vi "_CSMOFGV.vi"(6 "Operation":T7=enum."Get By Name", 7 "Allowed Messages (Empty For All)":string[](array[string]), 8 "Error In":errorcluster caption="error in (no error)", 9 "Mode":T1, 10 "Reference":string, 11 "Name (\"\" to Use UUID) In":string) -> (0 "error out":errorcluster, 1 "Boolean":bool, 3 "Array":T2[](array[typedef]))   [LabVIEW 2017, in "Communicable State Machine.lvlib"]
uses:
  Communicable State Machine.lvlib
  _CSMOFGVOPER.ctl
  _CSMObj.ctl
  _CSMObj-Info.ctl
  Typedef/_CSM_MODE.ctl
  _CSMObj-Refs.ctl
  _CSMObj-Data.ctl
  Typedef/_CSM_MSG_TYPE.ctl
  Priority Queue/Priority Queue.ctl
  Typedef/_Cross CSM State Data.ctl
  Typedef/_Cross CSM State Response.ctl
  Typedef/_CSM_Response Source Message.ctl
  Priority Queue/def-Data(LowPRI-Q).ctl
  _CSMObj-ModeData.ctl
  Typedef/_CSM Status Change Event Data.ctl
  Typedef/_CSM_List Module Scope.ctl
  Def-CSMOMgr.ctl
  ChangeFlag/ChangeFlag-Write.vi
  Utility/Random Change Flag.vi
  ChangeFlag/ChangeFlagDB.vi
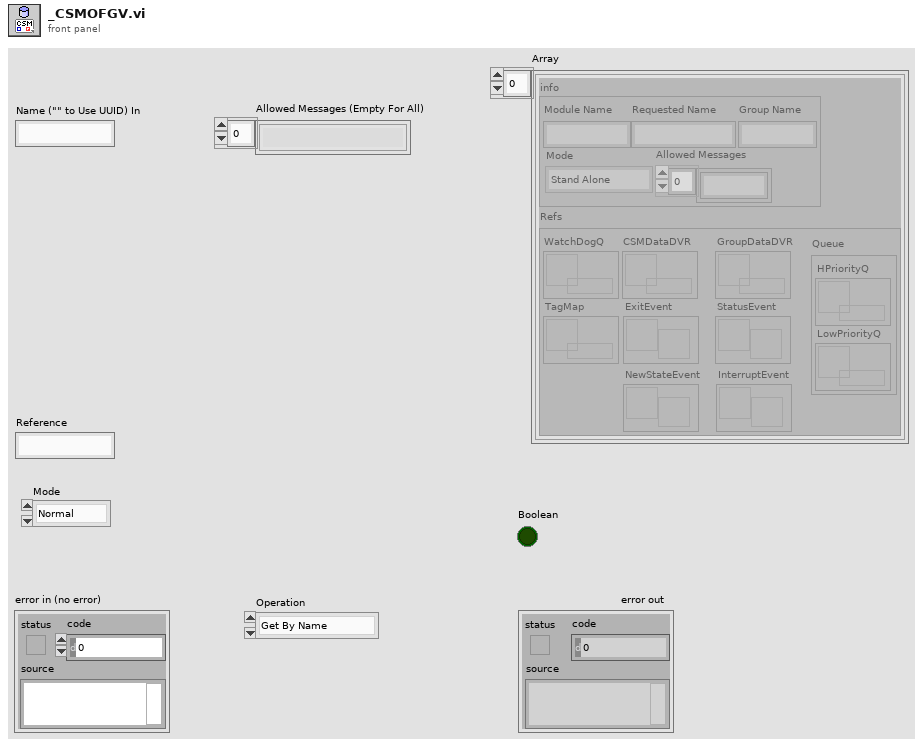
[diagram p1: front panel]
types:
  T1 = typedef "Communicable State Machine.lvlib/_CSM_List Module Scope.ctl" = enum16{"Normal", "System Only", "All"}
  T2 = typedef "Communicable State Machine.lvlib/_CSMObj.ctl" = cluster{"info":T3, "Refs":T5}
  T3 = typedef "Communicable State Machine.lvlib/_CSMObj-Info.ctl" = cluster{"Module Name":string, "Requested Name":string, "Group Name":string, "Mode":T4, "Allowed Messages":string[]}
  T4 = typedef "Communicable State Machine.lvlib/_CSM_MODE.ctl" = enum16{"Not Exist", "Stand Alone", "CSM", "Worker", "Worker Agent", "Chain Node", "Chain"}
  T5 = typedef "Communicable State Machine.lvlib/_CSMObj-Refs.ctl" = cluster{"WatchDogQ":refnum<queue>, "CSMDataDVR":refnum<data-value>, "Queue":T6, "GroupDataDVR":refnum<data-value>, "TagMap":refnum<data-value>, "ExitEvent":refnum<user-event>, "NewStateEvent":refnum<user-event>, "StatusEvent":refnum<user-event>, "InterruptEvent":refnum<user-event>}
  T6 = typedef "Communicable State Machine.lvlib/Priority Queue.ctl" = cluster{"HPriorityQ":refnum<queue>, "LowPriorityQ":refnum<queue>}
  T7 = typedef "Communicable State Machine.lvlib/_CSMOFGVOPER.ctl" = enum16{"Create If not Exist", "Get By Name", "List", "Check If Name Exists", "Release", "Module Status", "Create Status Event Handler", "Destroy Status Event Handler", "Clear Invalid Objs"}
  T8 = typedef "Communicable State Machine.lvlib/Def-CSMOMgr.ctl" = variant
  T9 = typedef "Communicable State Machine.lvlib/_CSMObj-ModeData.ctl" = cluster{"CSMDataDVR":refnum<data-value>[], "PriorityQueues":T6[], "Messages of Chain Nodes":cluster{"Module Name":string, "Allowed Messages":string[]}[], "Chain Message Mapping Map":variant, "SharedRegistryRules":string[]}
  T10 = cluster{"Module Name":string, "Allowed Messages":string[]}[]
  T11 = typedef "Communicable State Machine.lvlib/_CSMObj-Data.ctl" = cluster{"RemoteMessge?":bool, "error":errorcluster, "Return State":string, "Initialized":enum16{"Initializing", "Ready", "Exiting"}, "InternalRegistryRules":string[], "Return Msg Type":T12, "Current State":string, "Remaing JKISM Queue":string}
  T12 = typedef "Communicable State Machine.lvlib/_CSM_MSG_TYPE.ctl" = enum16{"Sync Message(-@)", "Async Message(->)", "Async without Response(->|)", "Async Response", "Broadcast(-><all>)", "Broadcast(-><status>)", "Broadcast(-><interrupt>)", "Append to JKISM States", "Append to JKISM States(High Priority)", "Broadcast(-><state>)", "<None>"}
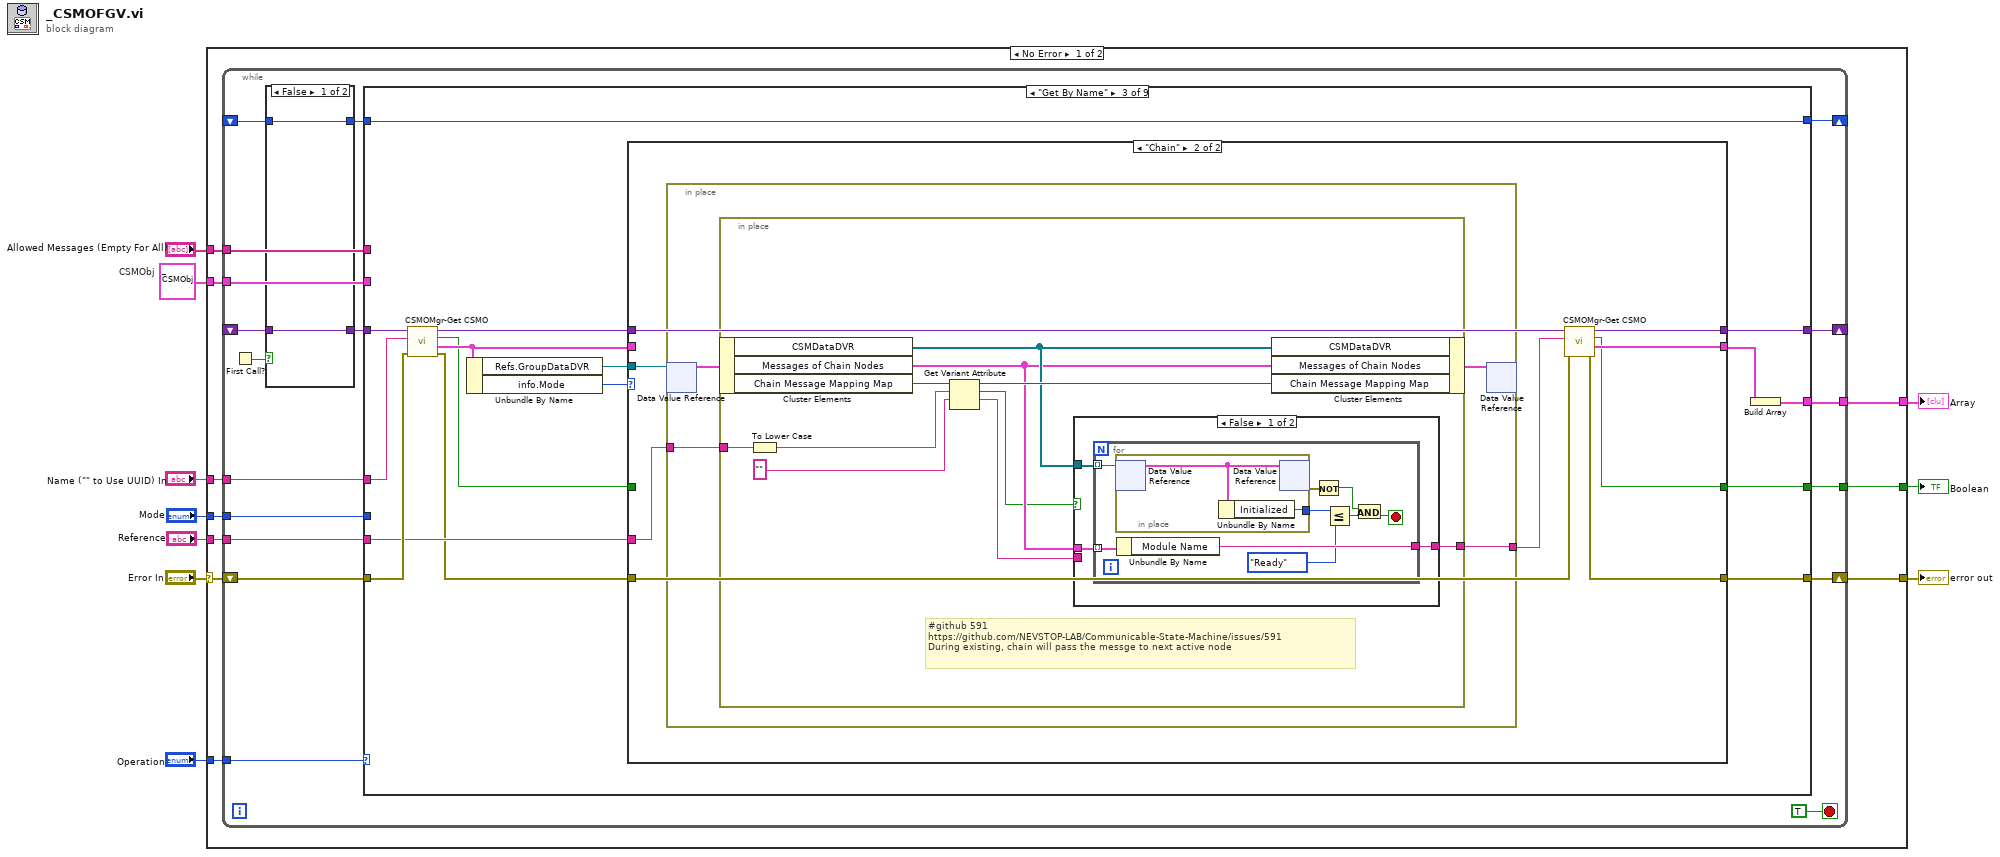
[diagram p0: block diagram]
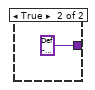
[diagram p2: hidden frame]
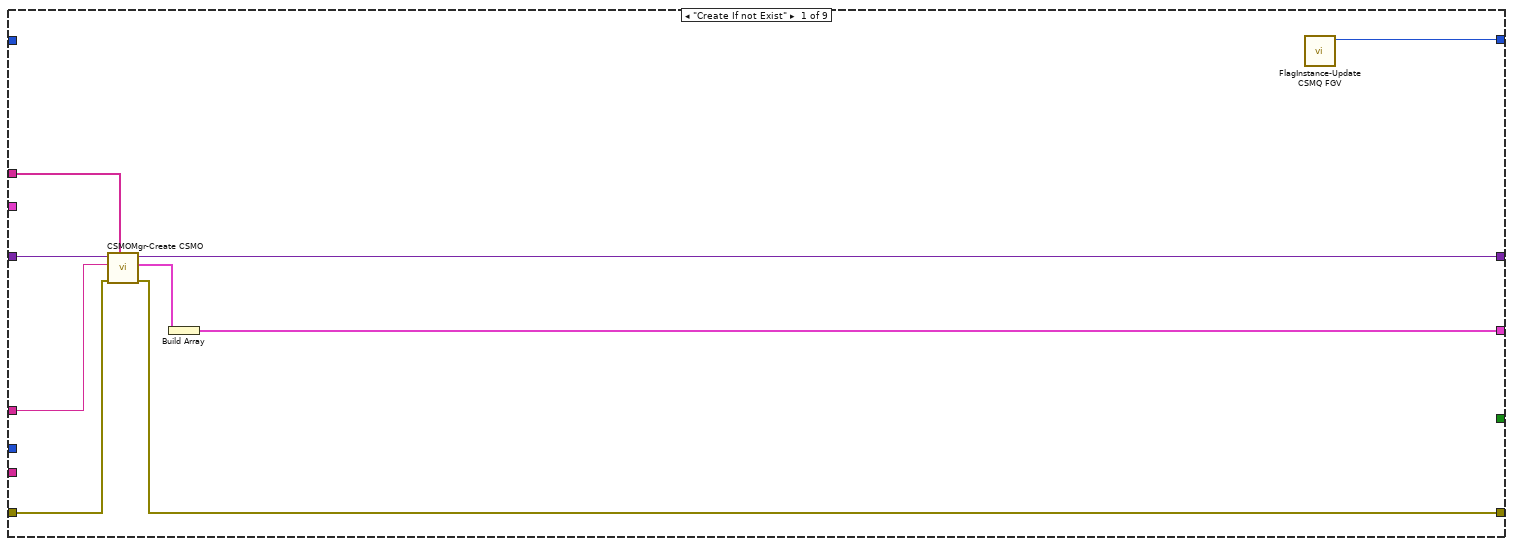
[diagram p3: hidden frame]
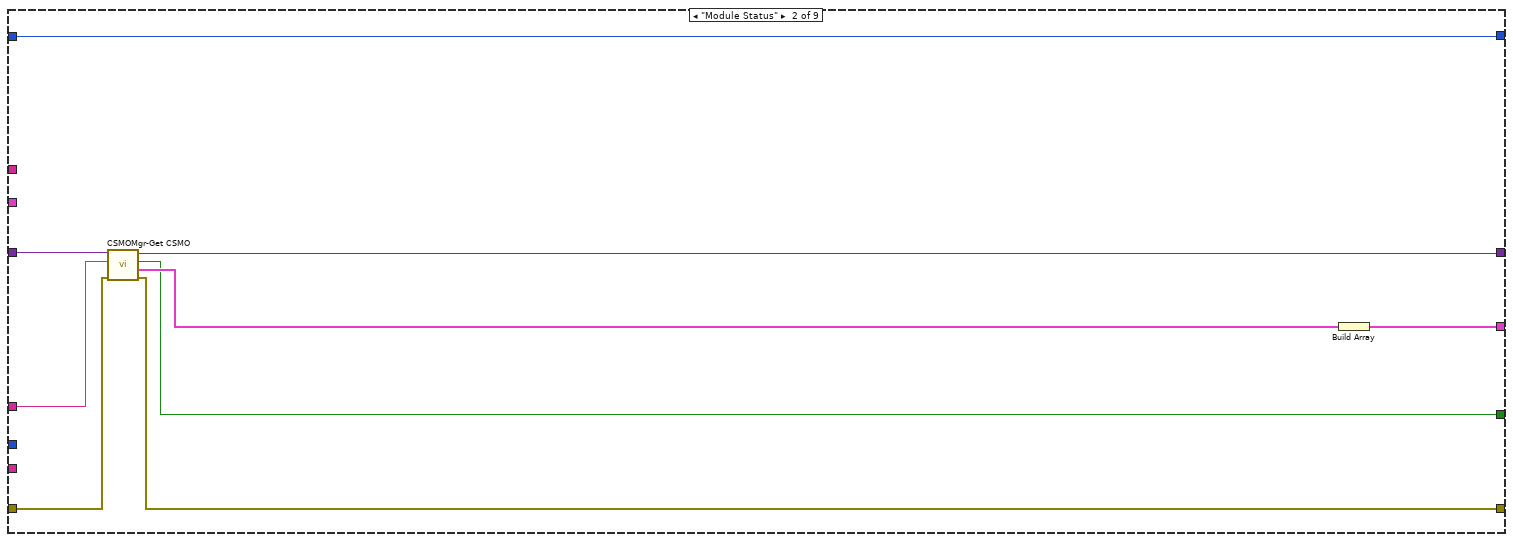
[diagram p4: hidden frame]
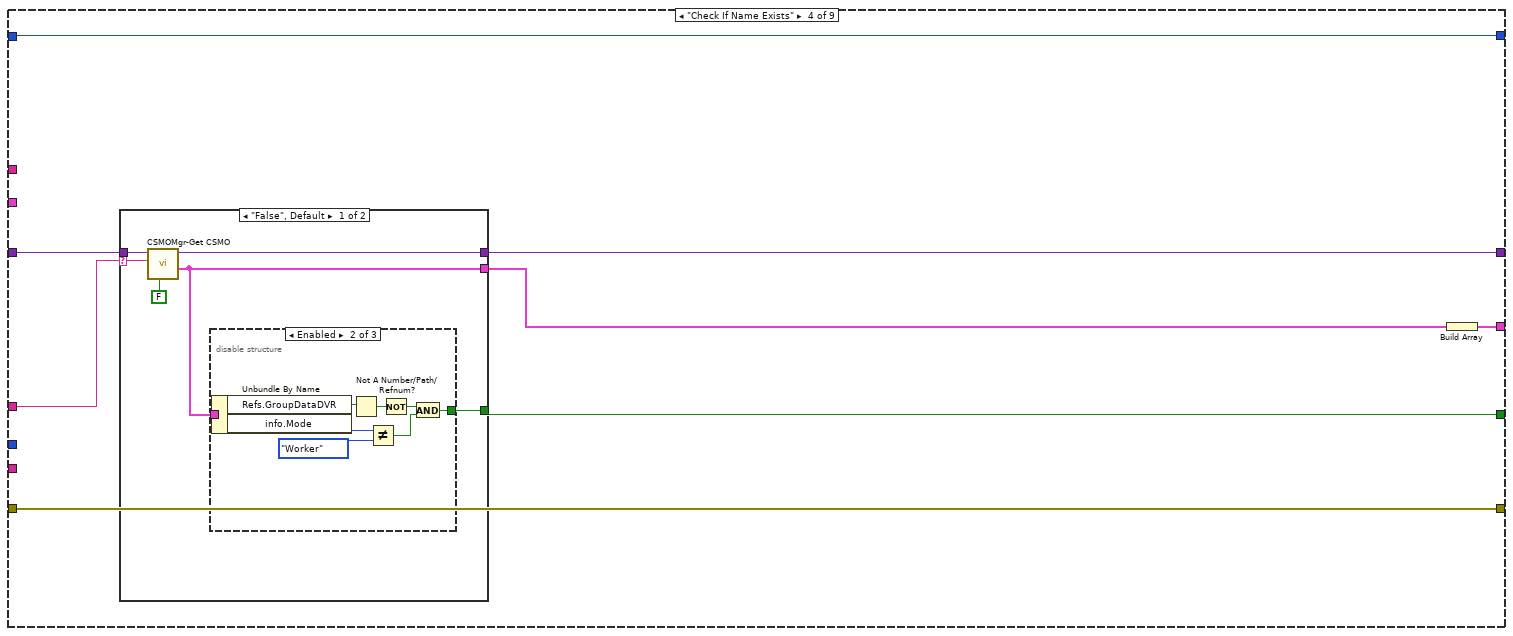
[diagram p7: hidden frame]
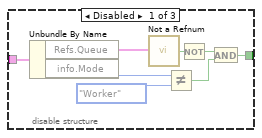
[diagram p8: hidden frame]
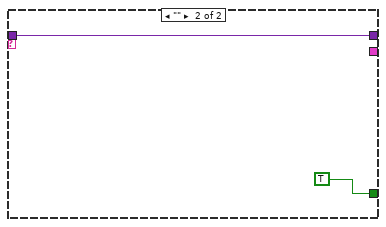
[diagram p10: hidden frame]
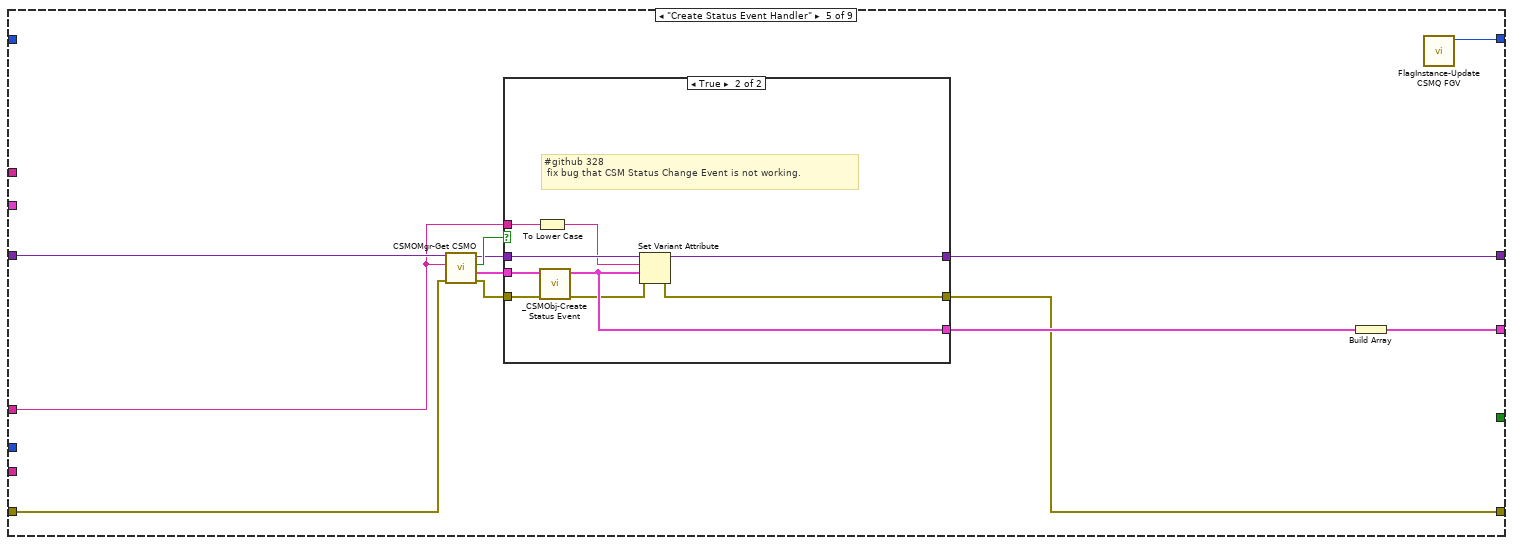
[diagram p11: hidden frame]
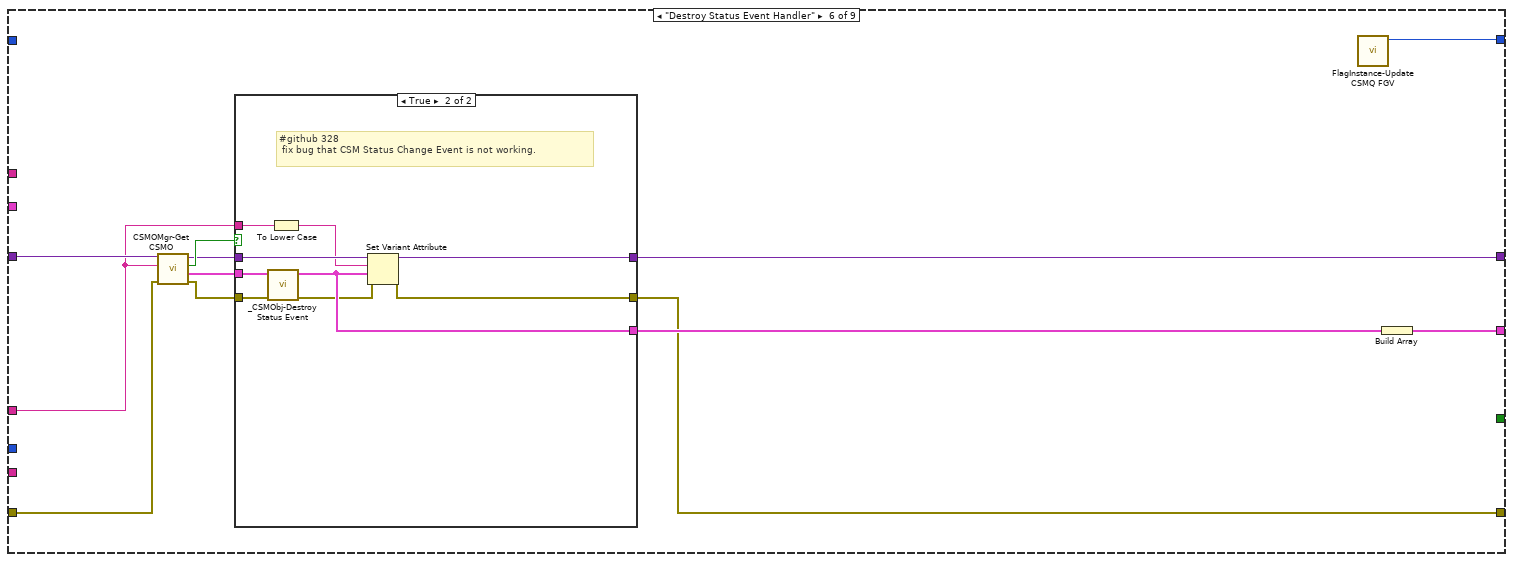
[diagram p13: hidden frame]
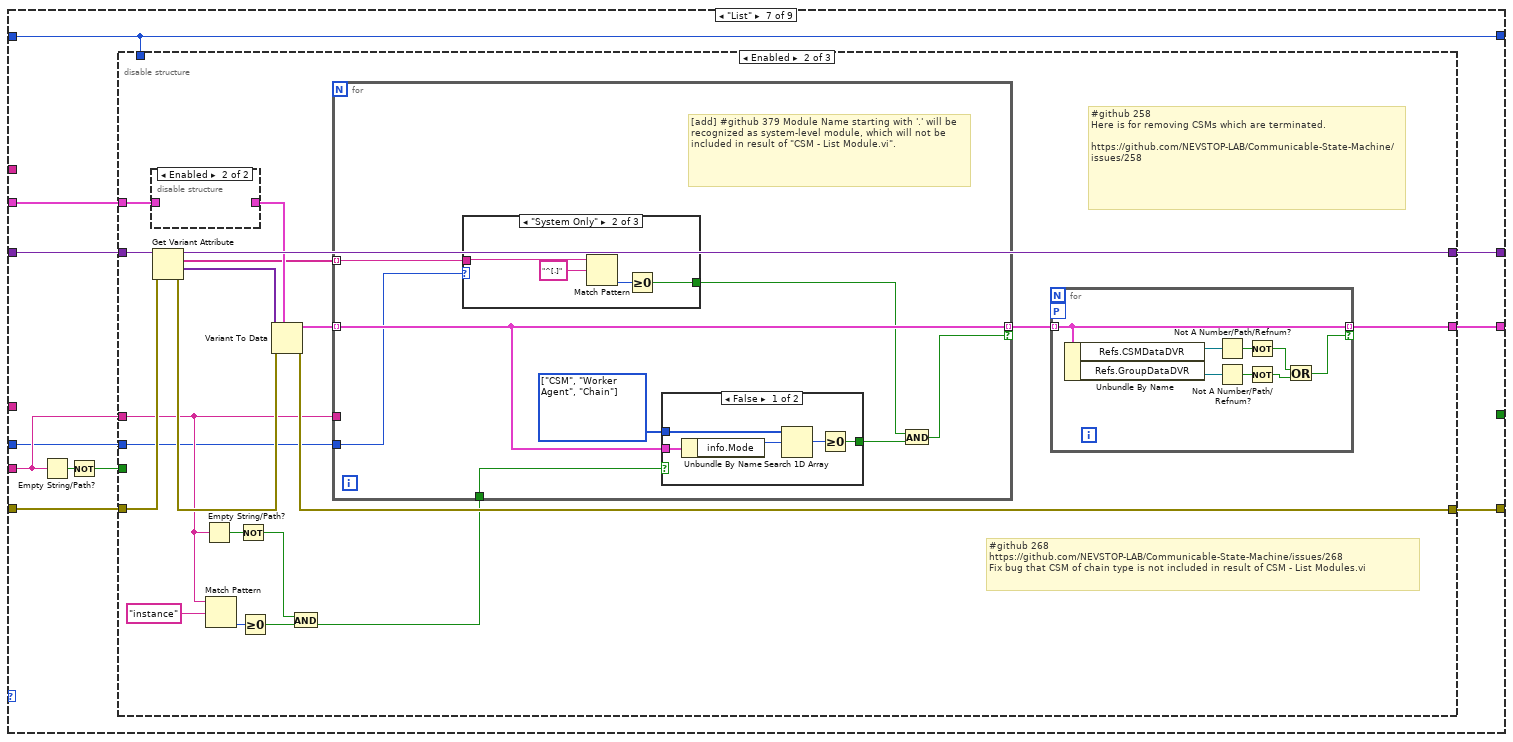
[diagram p15: hidden frame]
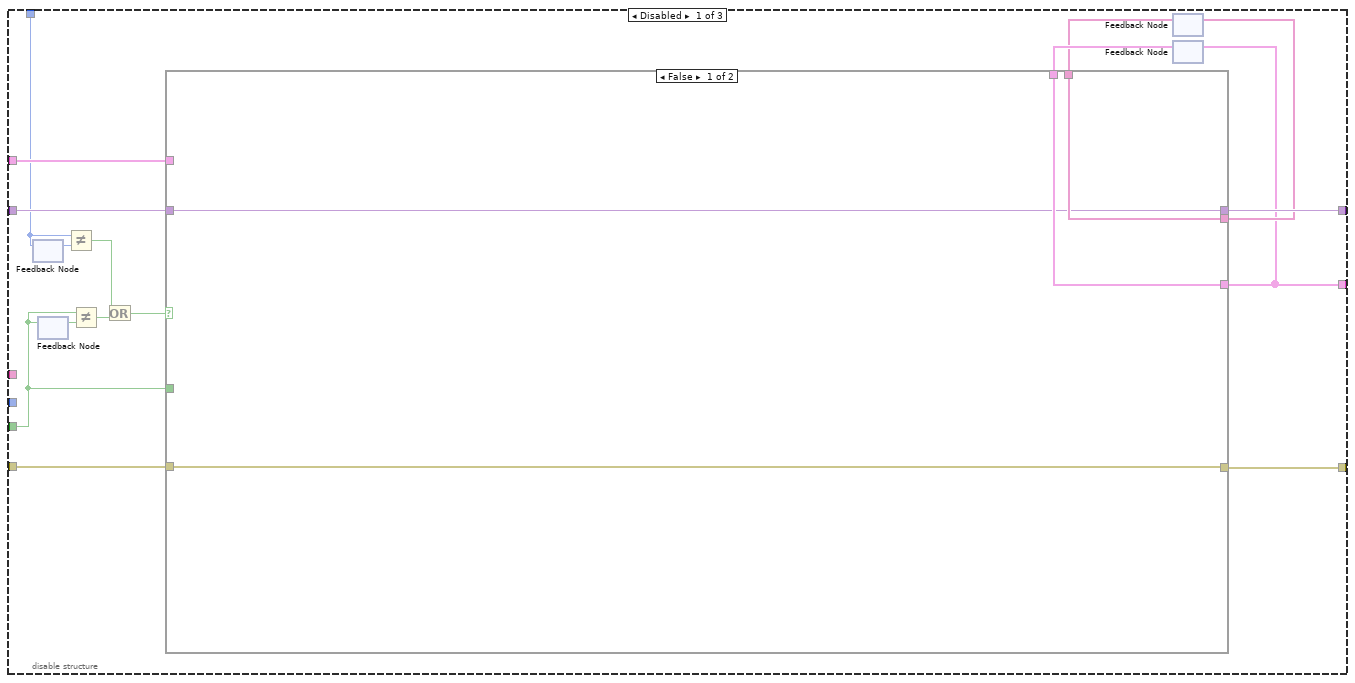
[diagram p16: hidden frame]
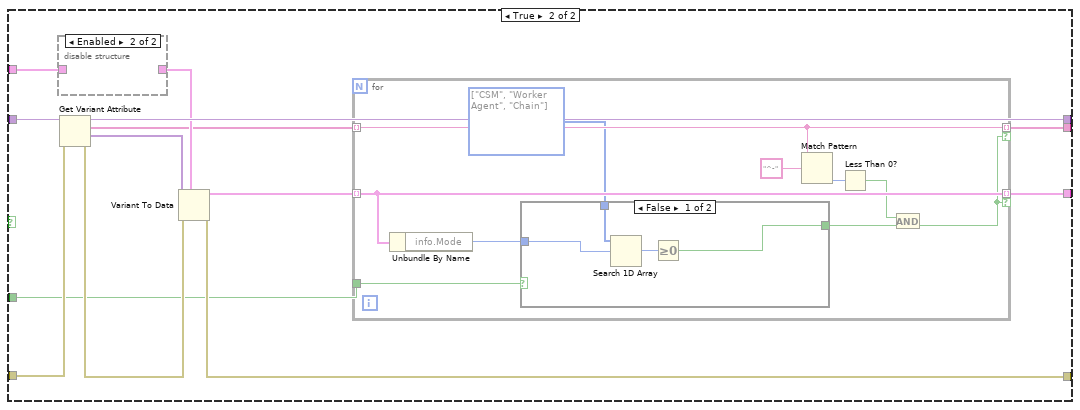
[diagram p17: hidden frame]
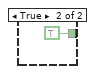
[diagram p18: hidden frame]
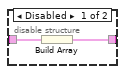
[diagram p19: hidden frame]
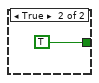
[diagram p20: hidden frame]
diagram:
  w6 = T2 {"info"={"Module Name"="", "Requested Name"="", "Group Name"="", "Mode"=enum."Stand Alone", "Allowed Messages"=[]}, "Refs"={"WatchDogQ"=refnum, "CSMDataDVR"=refnum, "Queue"={"HPriorityQ"=refnum, "LowPriorityQ"=refnum}, "GroupDataDVR"=refnum, "TagMap"=refnum, "ExitEvent"=refnum, "NewStateEvent"=refnum, "StatusEvent"=refnum, "InterruptEvent"=refnum}}  # CSMObj
  n1 = case shown="No Error" "Error In" {
    selector: "Error In" -> [w18 w351]
    tunnel: "Operation" -> [w20 _]
    tunnel: "Name (\"\" to Use UUID) In" -> [w19 _]
    tunnel: [w17 w351] -> w7
    tunnel: w6 -> [w16 _]
    tunnel: [w15 _] -> w5
    tunnel: [w14 _] -> w4
    tunnel: "Allowed Messages (Empty For All)" -> [w13 _]
    tunnel: "Reference" -> [w12 _]
    tunnel: "Mode" -> [w11 _]
    frame No Error {
      n2 = while {
        tunnel: w20 -> [w37]
        tunnel: w19 -> [w36]
        tunnel: [w35] -> w15
        shift-right: [w31] -> _
        shift-left: _ -> [w33]
        shift-right: [w29] -> w17
        shift-left: w18 -> [w30]
        tunnel: w16 -> [w28]
        tunnel: [w27] -> w14
        shift-right: [w26] -> _
        shift-left: _ -> [w24]
        tunnel: w13 -> [w23]
        tunnel: w12 -> [w22]
        tunnel: w11 -> [w21]
        stop <- TRUE stop-if-true
        n3 = First Call?() -> (First Call?: T/F=w34:bool)
        n4 = case shown="False" w34 {
          tunnel: [w40 T8 variant] -> w32
          tunnel: w33 -> [w40 _]
          tunnel: [w39 _] -> w25
          tunnel: w24 -> [w39 _]
          frame False {
          }
          frame True {
          }
        }
        n5 = case shown="\"Get By Name\"" w37 {
          tunnel: w36 -> [w43 w51 w71 w118 w160 w184 _ _ w348]
          tunnel: [w46 w56 w74 w122 w154 w178 w202 _ _] -> w35
          tunnel: w32 -> [w44 w59 w75 w119 w161 w185 w208 w323 w350]
          tunnel: [w50 w58 w67 w125 w156 w180 w207 w312 w347] -> w31
          tunnel: w30 -> [w47 w54 w72 w123 w153 w177 w205 w321 w349]
          tunnel: [w49 w53 w60 w123 w151 w175 w204 w320 w346] -> w29
          tunnel: w28 -> [_ _ _ _ _ _ w206 w322 _]
          tunnel: [_ w52 w61 w121 _ _ _ _ _] -> w27
          tunnel: w25 -> [_ w55 w73 w120 _ _ w203 w319 _]
          tunnel: [w42 w55 w73 w120 w150 w174 w203 w319 w345] -> w26
          tunnel: w23 -> [w45 _ _ _ _ _ _ _ _]
          tunnel: w22 -> [_ _ w65 _ _ _ w199 _ _]
          tunnel: w21 -> [_ _ _ _ _ _ w198 _ _]
          frame "Create If not Exist" {
            n6 = call "CSMOMgr-Create CSMO.vi"("Allowed Messages (Empty For All)"=w45, "error in (no error)"=w47, "Name (\"\" to Use UUID) In"=w43, "CSMOMgr"=w44) -> ("error out"=w49:errorcluster, "CSMO"=w48:T2, "CSMOMgr Out"=w50:T8)  [unwired: 5 in]
            n7 = Build Array(w48) -> (w46:T2[])
            n8 = call "FlagInstance-Update CSMQ FGV.vi"() -> ("New Random Change Flag"=w42:u64)  [unwired: 10 in, 1 out]
          }
          frame "Module Status" {
            n9 = call "CSMOMgr-Get CSMO.vi"("Error In"=w54, "Queue Name"=w51, "CSMOMgr"=w59) -> ("error out"=w53:errorcluster, "Values"=w57:T2, "Found"=w52:bool, "CSMOMgr Out"=w58:T8)  [unwired: 5 in]
            n10 = Build Array(w57) -> (w56:T2[])
          }
          frame "Get By Name" {
            n11 = call "CSMOMgr-Get CSMO.vi"("Error In"=w72, "Queue Name"=w71, "CSMOMgr"=w75) -> ("error out"=w63:errorcluster, "Values"=w69:T2, "Found"=w62:bool, "CSMOMgr Out"=w66:T8)  [unwired: 5 in]
            n12 = Unbundle By Name(w69) -> ("Refs.GroupDataDVR"=w64:refnum<data-value>, "info.Mode"=w70:T4)
            n13 = case shown="\"Chain\"" w70 {
              tunnel: w69 -> [w79 _]
              tunnel: [w79 w86] -> w68
              tunnel: [w78 w81] -> w67
              tunnel: w66 -> [w78 w82]
              tunnel: w65 -> [_ w87]
              tunnel: w64 -> [_ w88]
              tunnel: w63 -> [w76 w84]
              tunnel: w62 -> [w77 _]
              tunnel: [w77 w85] -> w61
              tunnel: [w76 w83] -> w60
              frame "Not Exist", Default {
              }
              frame "Chain" {
                n14 = in-place {
                  in-place-border: w87 -> [w90]
                  in-place-border: [w89] -> w80
                  n15 = in-place-dvr #1(w88) -> (w92:T9)  [unwired: 1 out]
                  n16 = in-place {
                    in-place-border: w90 -> [w100]
                    in-place-border: [w93] -> w89
                    # "#github 591\nhttps://github.com/NEVSTOP-LAB/Communicable-State-Machine/issues/591\nDuring existing, chain will pass the messge to next active node"
                    n17 = in-place-cluster #2(w92) -> ("CSMDataDVR"=w97:refnum<data-value>[], "Messages of Chain Nodes"=w96:T10, "Chain Message Mapping Map"=w102:variant)
                    n18 = To Lower Case(string=w100) -> (all lower case string=w98:string)
                    n19 = Get Variant Attribute(Variant=w102, name=w98, default value (empty Variant)="") -> (duplicate Variant=w101:variant, found=w95:bool, value=w94:string)  [unwired: 1 in, 1 out]
                    n20 = case shown="False" w95 {
                      tunnel: w97 -> [w105 _]
                      tunnel: w96 -> [w104 _]
                      tunnel: w94 -> [_ w117]
                      tunnel: [w103 w117] -> w93
                      frame False {
                        n21 = for {
                          tunnel: w105 -> [w114] mode=indexing
                          tunnel: w104 -> [w113] mode=indexing
                          tunnel: [w112] -> w103
                          stop <- w108 stop-if-true
                          n22 = in-place {
                            in-place-border: [w115] -> w111
                            n23 = in-place-dvr #3(w114) -> (w116:T11)  [unwired: 1 out]
                            n24 = Unbundle By Name(w116) -> ("Initialized"=w115:enum16{"Initializing", "Ready", "Exiting"})
                            n25 = in-place-dvr #3(w116) -> (w107:errorcluster)  [unwired: 1 out]
                          }
                          n26 = Unbundle By Name(w113) -> ("Module Name"=w112:string)
                          n27 = Not(x=w107) -> (.not. x?=w106:bool)
                          n28 = Less Or Equal?(x=w111, y=enum16{"Initializing", "Ready", "Exiting"}."Ready") -> (x <= y?=w109:bool)
                          n29 = And(x=w106, y=w109) -> (x .and. y?=w108:bool)
                        }
                      }
                      frame True {
                      }
                    }
                    n30 = in-place-cluster #2("CSMDataDVR"=w97, "Messages of Chain Nodes"=w96, "Chain Message Mapping Map"=w101) -> (w91:T9)
                  }
                  n31 = in-place-dvr #1(w91) -> ()  [unwired: 2 out]
                }
                n32 = call "CSMOMgr-Get CSMO.vi"("Error In"=w84, "Queue Name"=w80, "CSMOMgr"=w82) -> ("error out"=w83:errorcluster, "Values"=w86:T2, "Found"=w85:bool, "CSMOMgr Out"=w81:T8)  [unwired: 5 in]
              }
            }
            n33 = Build Array(w68) -> (w74:T2[])
          }
          frame "Check If Name Exists" {
            n34 = case shown="\"False\", Default" w118 {
              selector: w118 -> [w128 _]
              tunnel: w119 -> [w130 w149]
              tunnel: [w129 w149] -> w125
              tunnel: [w127 _] -> w124
              tunnel: [w131 TRUE] -> w121
              frame "False", Default {
                n35 = call "CSMOMgr-Get CSMO.vi"("GenError? (T)"=FALSE ("GenError?(T)"), "Queue Name"=w128, "CSMOMgr"=w130) -> ("Values"=w127:T2, "CSMOMgr Out"=w129:T8)  [unwired: 5 in, 2 out]
                n36 = disable-structure shown="Enabled" {
                  disable-tunnel: [w136 w144 _] -> w131
                  disable-tunnel: w127 -> [w132 w140 _]
                  frame Disabled {
                    n37 = Unbundle By Name(w132) -> ("Refs.Queue"=w139:T6, "info.Mode"=w135:T4)
                    n38 = call "Not a Refnum.vi"("Priority Queue.lvclass"=w139) -> ("NaN/Path/Refnum?"=w138:bool)  [unwired: 4 in]
                    n39 = Not Equal?(x=w135, y=_CSM_MODE."Worker") -> (x != y?=w133:bool)
                    n40 = Not(x=w138) -> (.not. x?=w137:bool)
                    n41 = And(x=w137, y=w133) -> (x .and. y?=w136:bool)
                  }
                  frame Enabled {
                    n42 = Unbundle By Name(w140) -> ("Refs.GroupDataDVR"=w147:refnum<data-value>, "info.Mode"=w143:T4)
                    n43 = Not A Number/Path/Refnum?(number/path/refnum=w147) -> (NaN/Path/Refnum?=w146:bool)
                    n44 = Not Equal?(x=w143, y=_CSM_MODE."Worker") -> (x != y?=w141:bool)
                    n45 = Not(x=w146) -> (.not. x?=w145:bool)
                    n46 = And(x=w145, y=w141) -> (x .and. y?=w144:bool)
                  }
                  frame Disabled {
                  }
                }
              }
              frame "" {
              }
            }
            n47 = Build Array(w124) -> (w122:T2[])
          }
          frame "Create Status Event Handler" {
            n48 = call "CSMOMgr-Get CSMO.vi"("Error In"=w153, "Queue Name"=w160, "CSMOMgr"=w161) -> ("error out"=w152:errorcluster, "Values"=w159:T2, "Found"=w158:bool, "CSMOMgr Out"=w157:T8)  [unwired: 5 in]
            n49 = case shown="True" w158 {
              tunnel: w159 -> [w163 w170]
              tunnel: w157 -> [w164 w173]
              tunnel: [w164 w172] -> w156
              tunnel: w160 -> [_ w171]
              tunnel: [w163 w169] -> w155
              tunnel: w152 -> [w162 w168]
              tunnel: [w162 w166] -> w151
              frame False {
              }
              frame True {
                # "#github 328\n fix bug that CSM Status Change Event is not working."
                n50 = To Lower Case(string=w171) -> (all lower case string=w165:string)
                n51 = call "_CSMObj-Create Status Event.vi"("Error In"=w168, "Values In"=w170) -> ("error out"=w167:errorcluster, "Values Out"=w169:T2)  [unwired: 8 in]
                n52 = Set Variant Attribute(Variant=w173, name=w165, value=w169, error in=w167) -> (Variant out=w172:T8, error out=w166:errorcluster)  [unwired: 1 out]
              }
            }
            n53 = Build Array(w155) -> (w154:T2[])
            n54 = call "FlagInstance-Update CSMQ FGV.vi"() -> ("New Random Change Flag"=w150:u64)  [unwired: 10 in, 1 out]
          }
          frame "Destroy Status Event Handler" {
            n55 = call "CSMOMgr-Get CSMO.vi"("Error In"=w177, "Queue Name"=w184, "CSMOMgr"=w185) -> ("error out"=w176:errorcluster, "Values"=w183:T2, "Found"=w182:bool, "CSMOMgr Out"=w181:T8)  [unwired: 5 in]
            n56 = case shown="True" w182 {
              tunnel: w183 -> [w187 w194]
              tunnel: w181 -> [w188 w197]
              tunnel: [w188 w196] -> w180
              tunnel: w184 -> [_ w195]
              tunnel: [w187 w193] -> w179
              tunnel: w176 -> [w186 w192]
              tunnel: [w186 w190] -> w175
              frame False {
              }
              frame True {
                # "#github 328\n fix bug that CSM Status Change Event is not working."
                n57 = call "_CSMObj-Destroy Status Event.vi"("Error In"=w192, "Values In"=w194) -> ("error out"=w191:errorcluster, "Values Out"=w193:T2)  [unwired: 8 in]
                n58 = To Lower Case(string=w195) -> (all lower case string=w189:string)
                n59 = Set Variant Attribute(Variant=w197, name=w189, value=w193, error in=w191) -> (Variant out=w196:T8, error out=w190:errorcluster)  [unwired: 1 out]
              }
            }
            n60 = call "FlagInstance-Update CSMQ FGV.vi"() -> ("New Random Change Flag"=w174:u64)  [unwired: 10 in, 1 out]
            n61 = Build Array(w179) -> (w178:T2[])
          }
          frame "List" {
            n62 = Empty String/Path?(string/path=w199) -> (empty?=w201:bool)
            n63 = Not(x=w201) -> (.not. x?=w200:bool)
            n64 = disable-structure shown="Enabled" {
              disable-tunnel: w208 -> [w224 w278 _]
              disable-tunnel: [w223 w277 _] -> w207
              disable-tunnel: w206 -> [w222 w276 _]
              disable-tunnel: w205 -> [w221 w275 _]
              disable-tunnel: [w220 w274 _] -> w204
              disable-tunnel: w203 -> [w218 _ _]
              disable-tunnel: [w212 w267 _] -> w202
              disable-tunnel: w200 -> [w209 _ _]
              disable-tunnel: w199 -> [_ w261 _]
              disable-tunnel: w198 -> [_ w259 _]
              frame Disabled {
                n65 = feedback #4() -> (w219:u64)  [unwired: 1 in]
                n66 = feedback-in #4(w218) -> ()
                n67 = feedback #5() -> (w217:bool)  [unwired: 1 in]
                n68 = feedback-in #5(w209) -> ()
                n69 = Not Equal?(x=w218, y=w219) -> (x != y?=w215:bool)
                n70 = Not Equal?(x=w209, y=w217) -> (x != y?=w216:bool)
                n71 = Or(x=w215, y=w216) -> (x .or. y?=w214:bool)
                n72 = feedback #6() -> (w210:string[])  [unwired: 1 in]
                n73 = feedback #7() -> (w211:T2[])  [unwired: 1 in]
                n74 = case shown="False" w214 {
                  tunnel: w224 -> [w226 w241]
                  tunnel: [w226 w240] -> w223
                  tunnel: w222 -> [_ w238]
                  tunnel: [w227 w234] -> w213
                  tunnel: [w228 w233] -> w212
                  tunnel: w221 -> [w225 w231]
                  tunnel: [w225 w230] -> w220
                  tunnel: w209 -> [_ w229]
                  tunnel: w211 -> [w228 _]
                  tunnel: w210 -> [w227 _]
                  frame False {
                  }
                  frame True {
                    n75 = disable-structure shown="Enabled" {
                      disable-tunnel: w238 -> [w258 _]
                      disable-tunnel: [w257 _] -> w237
                      frame Disabled {
                        n76 = Build Array(w258) -> (w257:T2[])
                      }
                      frame Enabled {
                      }
                    }
                    n77 = Get Variant Attribute(Variant=w241, error in=w231) -> (duplicate Variant=w240:variant, names=w235:string[], values=w239:variant[], error out=w232:errorcluster)  [unwired: 2 in]
                    n78 = Variant To Data(error in=w232, type=w237, Variant=w239) -> (data=w236:T2[], error out=w230:errorcluster)
                    n79 = for {
                      tunnel: w236 -> [w251] mode=indexing
                      tunnel: w235 -> [w246] mode=indexing
                      tunnel: [w246] -> w234 mode=indexing if=w247
                      tunnel: [w251] -> w233 mode=indexing if=w247
                      tunnel: w229 -> [w248]
                      w242 = T4[] [enum."CSM", enum."Worker Agent", enum."Chain"] items=["Not Exist", "Stand Alone", "CSM", "Worker", "Worker Agent", "Chain Node", "Chain"]
                      n80 = Unbundle By Name(w251) -> ("info.Mode"=w250:T4)
                      n81 = case shown="False" w248 {
                        tunnel: [w252 TRUE] -> w249
                        tunnel: w250 -> [w255 _]
                        tunnel: w242 -> [w254 _]
                        frame False {
                          n82 = Search 1D Array(1D array=w254, element=w255) -> (index of element=w253:i32)  [unwired: 1 in]
                          n83 = Greater Or Equal To 0?(x=w253) -> (x >= 0?=w252:bool)
                        }
                        frame True {
                        }
                      }
                      n84 = Match Pattern(string=w246, regular expression="^-") -> (offset past match=w244:i32)  [unwired: 1 in, 3 out]
                      n85 = Less Than 0?(x=w244) -> (x < 0?=w243:bool)
                      n86 = And(x=w243, y=w249) -> (x .and. y?=w247:bool)
                    }
                  }
                }
                n87 = feedback-in #6(w213) -> ()
                n88 = feedback-in #7(w212) -> ()
              }
              frame Enabled {
                # "#github 268\nhttps://github.com/NEVSTOP-LAB/Communicable-State-Machine/issues/268\nFix bug that CSM of chain type is not included in result of CSM - List Modules.vi"
                # "#github 258\nHere is for removing CSMs which are terminated.\n\nhttps://github.com/NEVSTOP-LAB/Communicable-State-Machine/issues/258"
                n89 = disable-structure shown="Enabled" {
                  disable-tunnel: w276 -> [w311 _]
                  disable-tunnel: [w310 _] -> w272
                  frame Disabled {
                    n90 = Build Array(w311) -> (w310:T2[])
                  }
                  frame Enabled {
                  }
                }
                n91 = Get Variant Attribute(Variant=w278, error in=w275) -> (duplicate Variant=w277:variant, names=w270:string[], values=w273:variant[], error out=w269:errorcluster)  [unwired: 2 in]
                n92 = Empty String/Path?(string/path=w261) -> (empty?=w262:bool)
                n93 = Match Pattern(string=w261, regular expression="instance") -> (offset past match=w265:i32)  [unwired: 1 in, 3 out]
                n94 = Not(x=w262) -> (.not. x?=w260:bool)
                n95 = Greater Or Equal To 0?(x=w265) -> (x >= 0?=w264:bool)
                n96 = Variant To Data(error in=w269, type=w272, Variant=w273) -> (data=w271:T2[], error out=w274:errorcluster)
                n97 = And(x=w260, y=w264) -> (x .and. y?=w263:bool)
                n98 = for {
                  tunnel: w271 -> [w294] mode=indexing
                  tunnel: w270 -> [w291] mode=indexing
                  tunnel: [w294] -> w268 mode=indexing if=w292
                  tunnel: w261 -> [_]
                  tunnel: w263 -> [w288]
                  tunnel: w259 -> [w287]
                  w289 = T4[] [enum."CSM", enum."Worker Agent", enum."Chain"] items=["Not Exist", "Stand Alone", "CSM", "Worker", "Worker Agent", "Chain Node", "Chain"]
                  # "[add] #github 379 Module Name starting with '.' will be recognized as system-level module, which will not be included in result of \"CSM - List Module.vi\"."
                  n99 = case shown="\"System Only\"" w287 {
                    tunnel: w291 -> [w304 w308 _]
                    tunnel: [w301 w305 TRUE] -> w290
                    frame "Normal" {
                      n100 = Match Pattern(string=w304, regular expression="^[.]") -> (offset past match=w302:i32)  [unwired: 1 in, 3 out]
                      n101 = Less Than 0?(x=w302) -> (x < 0?=w301:bool)
                    }
                    frame "System Only" {
                      n102 = Match Pattern(string=w308, regular expression="^[.]") -> (offset past match=w306:i32)  [unwired: 1 in, 3 out]
                      n103 = Greater Or Equal To 0?(x=w306) -> (x >= 0?=w305:bool)
                    }
                    frame "All" {
                    }
                  }
                  n104 = case shown="False" w288 {
                    tunnel: w294 -> [w299 _]
                    tunnel: [w297 TRUE] -> w293
                    tunnel: w289 -> [w296 _]
                    frame False {
                      n105 = Unbundle By Name(w299) -> ("info.Mode"=w298:T4)
                      n106 = Search 1D Array(1D array=w296, element=w298) -> (index of element=w295:i32)  [unwired: 1 in]
                      n107 = Greater Or Equal To 0?(x=w295) -> (x >= 0?=w297:bool)
                    }
                    frame True {
                    }
                  }
                  n108 = And(x=w290, y=w293) -> (x .and. y?=w292:bool)
                }
                n109 = for {
                  tunnel: w268 -> [w279] mode=indexing
                  tunnel: [w279] -> w267 mode=indexing if=w285
                  workers-P: _ -> [_]
                  n110 = Unbundle By Name(w279) -> ("Refs.CSMDataDVR"=w282:refnum<data-value>, "Refs.GroupDataDVR"=w281:refnum<data-value>)
                  n111 = Not A Number/Path/Refnum?(number/path/refnum=w282) -> (NaN/Path/Refnum?=w286:bool)
                  n112 = Not A Number/Path/Refnum?(number/path/refnum=w281) -> (NaN/Path/Refnum?=w283:bool)
                  n113 = Not(x=w286) -> (.not. x?=w284:bool)
                  n114 = Not(x=w283) -> (.not. x?=w280:bool)
                  n115 = Or(x=w284, y=w280) -> (x .or. y?=w285:bool)
                }
              }
              frame Disabled {
              }
            }
          }
          frame "Clear Invalid Objs" {
            n116 = disable-structure shown="Enabled" {
              disable-tunnel: w322 -> [w344 _]
              disable-tunnel: [w343 _] -> w317
              frame Disabled {
                n117 = Build Array(w344) -> (w343:T2[])
              }
              frame Enabled {
              }
            }
            n118 = Get Variant Attribute(Variant=w323, error in=w321) -> (duplicate Variant=w313:variant, names=w315:string[], values=w318:variant[], error out=w314:errorcluster)  [unwired: 2 in]
            n119 = Variant To Data(error in=w314, type=w317, Variant=w318) -> (data=w316:T2[], error out=w320:errorcluster)
            n120 = for {
              tunnel: w316 -> [w327] mode=indexing
              tunnel: w315 -> [w324] mode=indexing
              shift-right: [w326] -> w312
              shift-left: w313 -> [w325]
              (unwired) _CSM_MODE."Not Exist" ("Mode")
              w328 = T4[] [enum."CSM", enum."Worker Agent", enum."Chain"] items=["Not Exist", "Stand Alone", "CSM", "Worker", "Worker Agent", "Chain Node", "Chain"]
              n121 = Unbundle By Name(w327) -> ("info.Mode"=w329:T4)
              n122 = case shown="Default" w329 {
                tunnel: w328 -> [_]
                tunnel: w327 -> [w338]
                tunnel: [w334] -> w326
                tunnel: w325 -> [w335]
                tunnel: w324 -> [w333]
                frame Default {
                  n123 = Unbundle By Name(w338) -> ("Refs.CSMDataDVR"=w337:refnum<data-value>, "Refs.GroupDataDVR"=w336:refnum<data-value>)
                  n124 = Not A Number/Path/Refnum?(number/path/refnum=w337) -> (NaN/Path/Refnum?=w332:bool)
                  n125 = Not A Number/Path/Refnum?(number/path/refnum=w336) -> (NaN/Path/Refnum?=w331:bool)
                  n126 = Or(x=w332, y=w331) -> (x .or. y?=w330:bool)
                  n127 = case shown="True" w330 {
                    tunnel: w335 -> [w339 w342]
                    tunnel: [w339 w341] -> w334
                    tunnel: w333 -> [_ w340]
                    frame False {
                    }
                    frame True {
                      n128 = Delete Variant Attribute(6:w340, 7:w342) -> (3:w341:variant)  [unwired: 1 in, 2 out]
                    }
                  }
                }
              }
            }
          }
          frame "Release" {
            n129 = call "CSMOMgr-Delete CSMO.vi"("Error In"=w349, "Queue Name"=w348, "CSMOMgr"=w350) -> ("error out"=w346:errorcluster, "CSMOMgr Out"=w347:T8)  [unwired: 6 in, 1 out]
            n130 = call "FlagInstance-Update CSMQ FGV.vi"() -> ("New Random Change Flag"=w345:u64)  [unwired: 10 in, 1 out]
          }
        }
      }
    }
    frame Error {
    }
  }
  "error out" <- w7
  "Array" <- w5
  "Boolean" <- w4
